vi "Write DAT (1D).vi"(4 "Append (0=F)":i32, 6 "Comments":string, 8 "error in":errorcluster, 9 "Data":dbl[](array[numeric]), 10 "Headers":string[](array[string]), 11 "path":path) -> (0 "error out":errorcluster, 3 "new file path":path)   [LabVIEW 2019, in "LV-Data.DAT.lvclass"]
uses:
  LV-Data.DAT.lvclass
  <vilib>/Utility/file.llb/Write Delimited Spreadsheet (string).vi
panel:
  out "appended array":string[][](array[string])
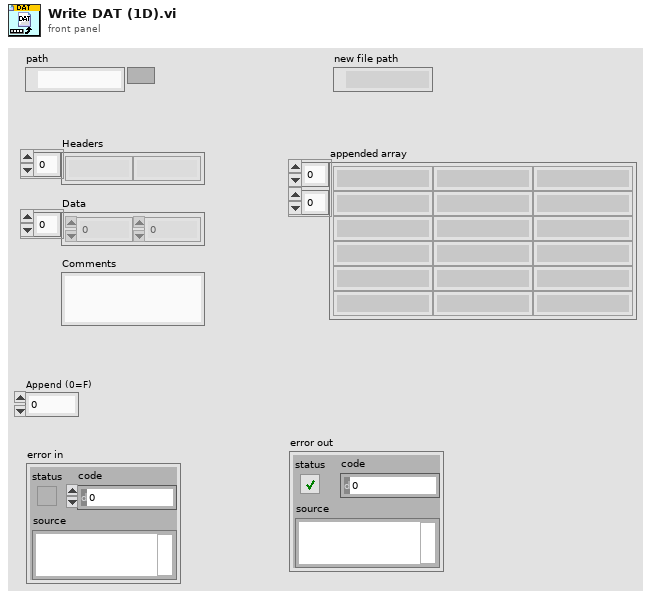
[diagram p1: front panel]
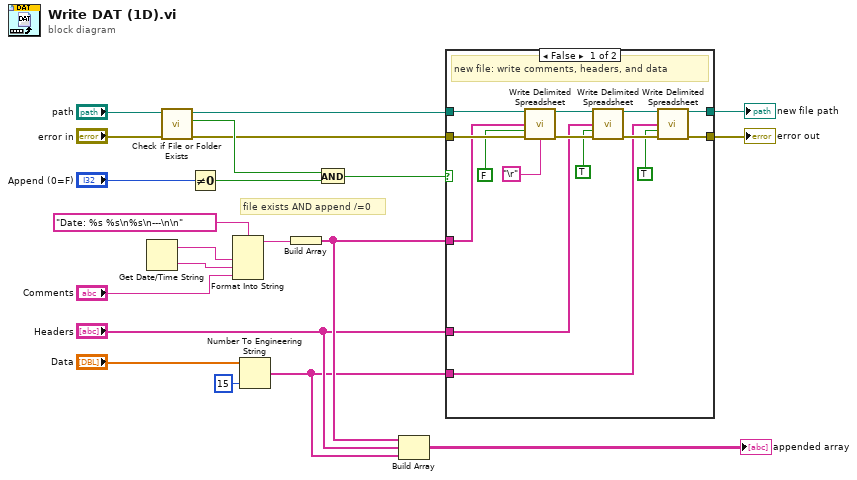
[diagram p0: block diagram]
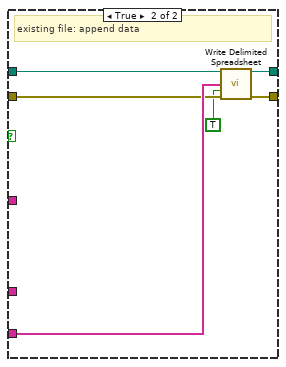
[diagram p2: hidden frame]
diagram:
  # "file exists AND append /=0"
  n1 = Get Date/Time String() -> (date string=w6:string, time string=w7:string)  [unwired: 3 out]
  n2 = call <vilib>:"Check if File or Folder Exists.vi"("error in (no error)"="error in", "path"="path") -> ("error out"=w8:errorcluster, "file or folder exists?"=w14:bool, "dup path"=w9:path)  [unwired: 7 in]
  n3 = Not Equal To 0?(x="Append (0=F)") -> (x != 0?=w13:bool)
  n4 = Format Into String(format string="Date: %s %s\n%s\n---\n\n", w6, w7, "Comments") -> (resulting string=w3:string)  [unwired: 2 in, 1 out]
  n5 = Number To Engineering String(2:i16 15 ("precision (6)"), 4:"Data") -> (0:w1:string[])  [unwired: 2 out]
  n6 = Build Array(w3) -> (w15:string[])
  n7 = And(x=w14, y=w13) -> (x .and. y?=w12:bool)
  n8 = Build Array(w15, "Headers", w1) -> (→"appended array":string[][])
  n9 = case shown="False" w12 {
    tunnel: w15 -> [w31 _]
    tunnel: [w27 w39] -> w19
    tunnel: w1 -> [w25 w41]
    tunnel: w9 -> [w36 w42]
    tunnel: w8 -> [w35 w40]
    tunnel: [w26 w38] -> w18
    tunnel: "Headers" -> [w28 _]
    frame False {
      # "new file: write comments, headers, and data"
      n10 = call-poly <vilib>:"Write Delimited Spreadsheet.vi"("file path (dialog if empty)"=w36, "1D data"=w31, "append to file? (new file:F)"=FALSE, "error in (no error)"=w35, "delimiter (\\t)"="\r") -> ("new file path (Not A Path if cancelled)"=w33:path, "error out"=w34:errorcluster)  [unwired: 9 in]
      n11 = call-poly <vilib>:"Write Delimited Spreadsheet.vi"("file path (dialog if empty)"=w33, "1D data"=w28, "append to file? (new file:F)"=TRUE, "error in (no error)"=w34) -> ("new file path (Not A Path if cancelled)"=w29:path, "error out"=w30:errorcluster)  [unwired: 10 in]
      n12 = call-poly <vilib>:"Write Delimited Spreadsheet.vi"("file path (dialog if empty)"=w29, "1D data"=w25, "append to file? (new file:F)"=TRUE, "error in (no error)"=w30) -> ("new file path (Not A Path if cancelled)"=w27:path, "error out"=w26:errorcluster)  [unwired: 10 in]
    }
    frame True {
      # "existing file: append data"
      n13 = call-poly <vilib>:"Write Delimited Spreadsheet.vi"("file path (dialog if empty)"=w42, "1D data"=w41, "append to file? (new file:F)"=TRUE, "error in (no error)"=w40) -> ("new file path (Not A Path if cancelled)"=w39:path, "error out"=w38:errorcluster)  [unwired: 10 in]
    }
  }
  "new file path" <- w19
  "error out" <- w18
